vi "run.get.multiple.vi"(8 "error in":errorcluster, 10 "rid(s)":string[](array[string]), 11 "Nominal Client in":refnum<class "Nominal Client.lvclass">) -> (0 "error out":errorcluster, 2 "Runs":refnum<class "Run.lvclass">[](array[class]), 3 "Nominal Client out":refnum<class "Nominal Client.lvclass">)   [LabVIEW 2020, in "Nominal Client.lvclass"]
doc: "Fetches details about the run in question based on its RID."
uses:
  Nominal Client.lvclass
  Run/Run.lvclass
  49411445-db77-4211-b7bb-06afe579b778.vi
  <vilib>/JDP Science/JSONtext/Variant to JSON Text.vi
  <vilib>/JDP Science/JSONtext/LVClass Serializer/JSONtext LVClass Serializer.lvclass
  Nominal Client.lvclass/Nominal Client.ctl
  <vilib>/JDP Science/JSONtext/JSONtext.lvlib
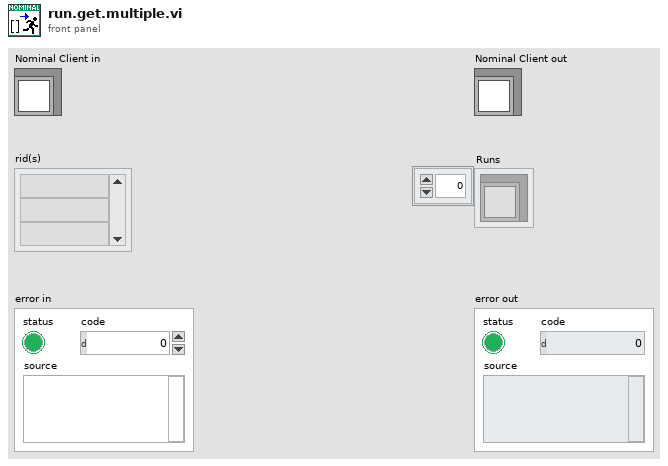
[diagram p1: front panel]
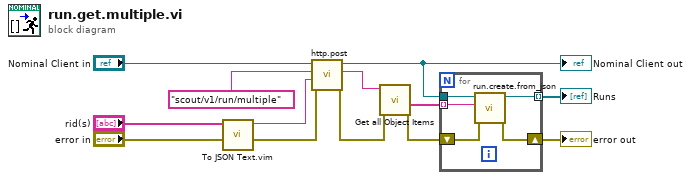
[diagram p0: block diagram]
diagram:
  n1 = call "To JSON Text.vim"("error in (no error)"="error in", "Anything"="rid(s)") -> ("error out"=w9:errorcluster, "<JSON>"=w8:string)  [unwired: 8 in]
  n2 = call "http.post.vi"("error in"=w9, "Request body"=w8, "Path"="scout/v1/run/multiple", "Nominal Client in"="Nominal Client in") -> ("error out"=w2:errorcluster, "Response"=w7:string, "Nominal Client out"=w1:refnum<class "Nominal Client.lvclass">)  [unwired: 4 in, 1 out]
  "Nominal Client out" <- w1
  n3 = call <vilib>:"Get all Object Items.vi"("error in (no error)"=w2, "JSON"=w7) -> ("error out"=w3:errorcluster, "<JSON>"=w6:string[])  [unwired: 6 in, 2 out]
  n4 = for {
    tunnel: w6 -> [w18] mode=indexing
    tunnel: [w15] -> w4 mode=indexing
    shift-right: [w16] -> w5
    shift-left: w3 -> [w17]
    tunnel: w1 -> [w14]
    n5 = call "run.create.from_json.vi"("error in"=w17, "JSON"=w18, "Nominal Client"=w14) -> ("error out"=w16:errorcluster, "Run out"=w15:refnum<class "Run.lvclass">)  [unwired: 7 in]
  }
  "error out" <- w5
  "Runs" <- w4
